vi "UI_Tile_Hit.vi"(0 "X":i32, 5 "Y":i32, 11 "error in":errorcluster) -> (4 "Channel Index":i32=-1, 15 "error out":errorcluster)   [LabVIEW 2026]
doc: "클릭 좌표 -> 채널 번호(0~127), 타일 밖이면 -1."
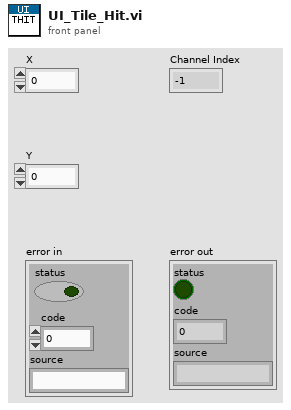
[diagram p1: front panel]
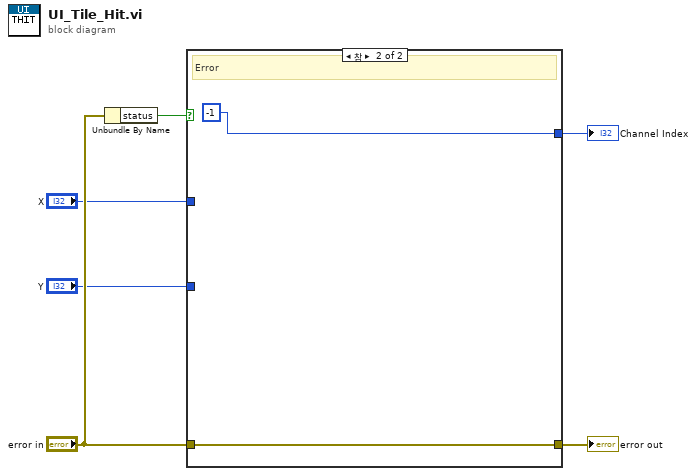
[diagram p0: block diagram]
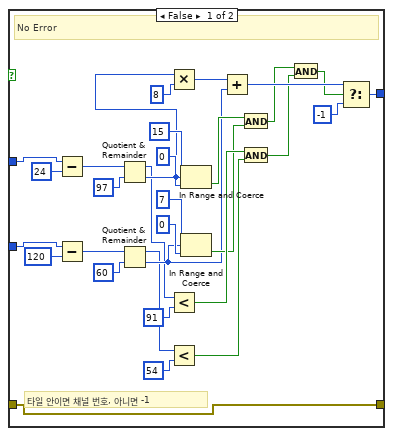
[diagram p2: hidden frame]
diagram:
  n1 = Unbundle By Name("error in") -> ("status"=w4:bool)
  n2 = case shown="참" w4 {
    tunnel: "X" -> [w7 _]
    tunnel: "Y" -> [w8 _]
    tunnel: "error in" -> [w9 w38]
    tunnel: [w9 w38] -> w6
    tunnel: [w37 -1] -> w5
    frame False {
      # "타일 안이면 채널 번호, 아니면 -1"
      # "No Error"
      n3 = Subtract(x=w7, y=24) -> (x-y=w11:i32)
      n4 = Subtract(x=w8, y=120) -> (x-y=w13:i32)
      n5 = Quotient & Remainder(x=w11, y=97) -> (x-y*floor(x/y)=w15:i32, floor(x/y)=w16:i32)
      n6 = Quotient & Remainder(x=w13, y=60) -> (x-y*floor(x/y)=w18:i32, floor(x/y)=w19:i32)
      n7 = Multiply(x=w16, y=8) -> (x*y=w34:i32)
      n8 = Less?(x=w15, y=91) -> (x < y?=w28:bool)
      n9 = Less?(x=w18, y=54) -> (x < y?=w30:bool)
      n10 = In Range and Coerce(upper limit=15, x=w16, lower limit=0) -> (In Range?=w22:bool)  [unwired: 1 out]
      n11 = In Range and Coerce(upper limit=7, x=w19, lower limit=0) -> (In Range?=w25:bool)  [unwired: 1 out]
      n12 = Add(x=w34, y=w19) -> (x+y=w35:i32)
      n13 = And(x=w22, y=w25) -> (x .and. y?=w26:bool)
      n14 = And(x=w28, y=w30) -> (x .and. y?=w31:bool)
      n15 = And(x=w26, y=w31) -> (x .and. y?=w32:bool)
      n16 = Select(t=w35, s=w32, f=-1) -> (s? t:f=w37:i32)
    }
    frame True {
      # "Error"
    }
  }
  "Channel Index" <- w5
  "error out" <- w6
